vi "optical_1.vi"() -> ()   [LabVIEW 2025]
panel:
  out "Optical saving error":errorcluster
  out "Times between Frames":u32
  in  "STOP ACQUISITION":bool
  out "Optical Frame Out":string
  out "Optical Preview":T1(plugin-control)
  in  "Output Folder":path
  # "Thermal Record"
  # "(Enter \"28\")"
  # "^ append to base data folder \"...\\test_n\\raw\" for nth recording"
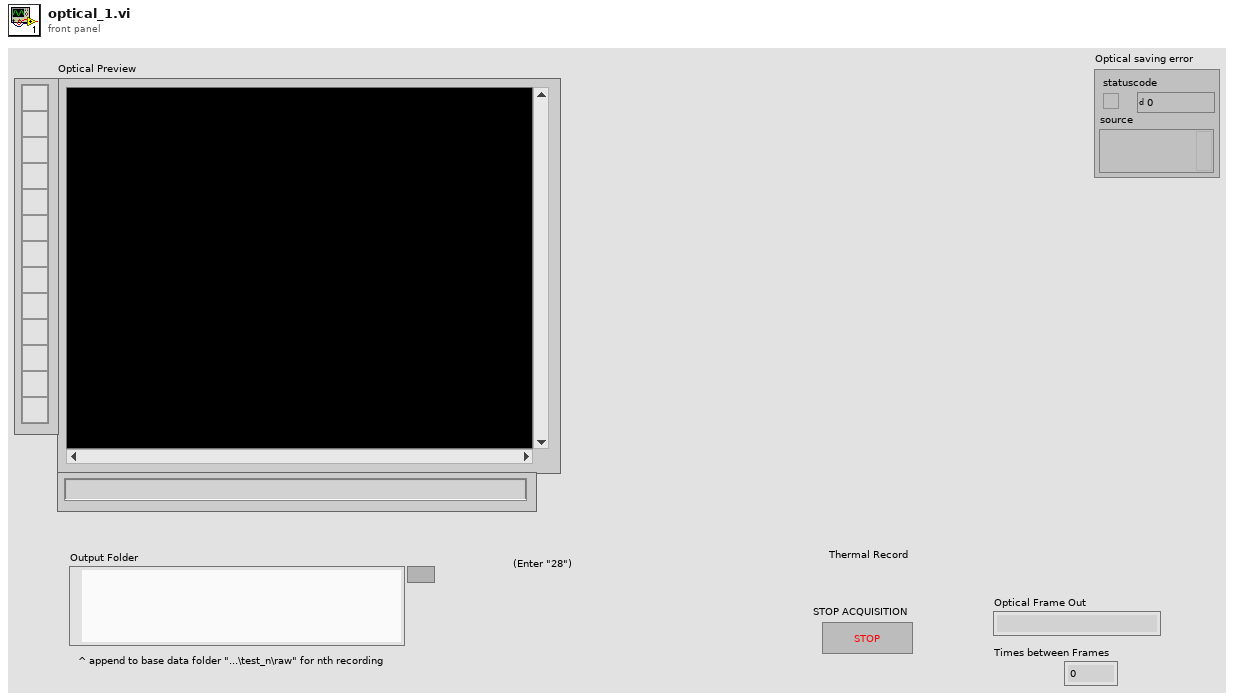
[diagram p1: front panel]
types:
  T1 = typedef "IMAQ Image.ctl" = refnum<image>
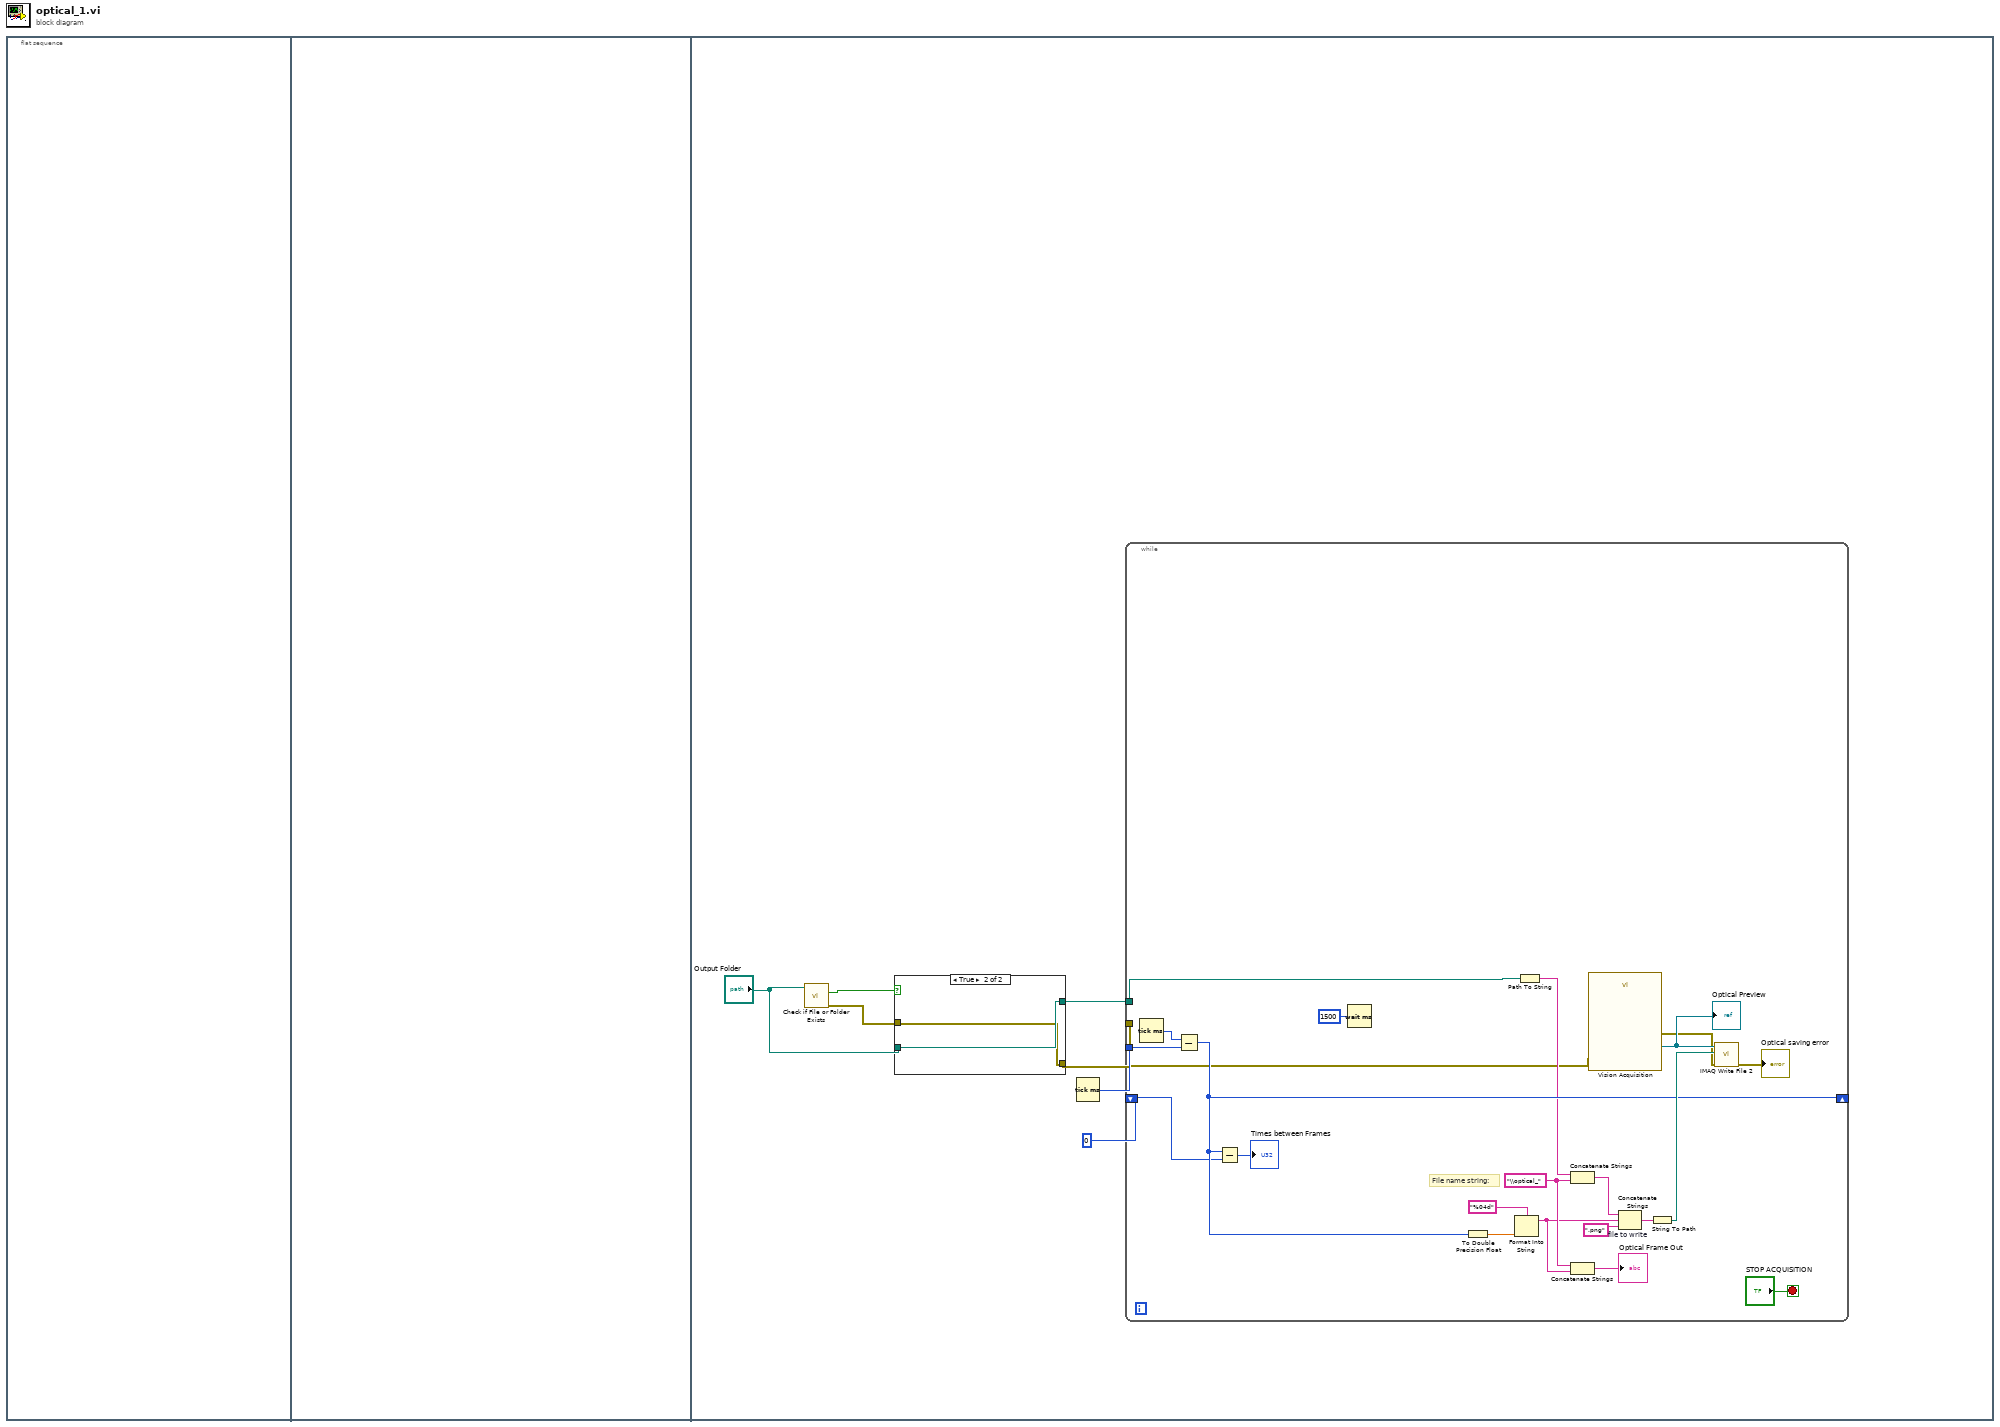
[diagram p0: block diagram]
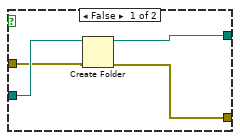
[diagram p2: hidden frame]
diagram:
  n1 = flat-sequence {
    frame #0 {
    }
    frame #1 {
    }
    frame #2 {
      n2 = call <vilib>:"Check if File or Folder Exists.vi"("path"="Output Folder") -> ("error out"=w2:errorcluster, "file or folder exists?"=w5:bool)  [unwired: 8 in, 1 out]
      n3 = case shown="True" w5 {
        tunnel: "Output Folder" -> [w11 w13]
        tunnel: [w10 w13] -> w3
        tunnel: w2 -> [w9 w12]
        tunnel: [w8 w12] -> w1
        frame False {
          n4 = Create Folder(path (use dialog)=w11, error in=w9) -> (created path=w10:path, error out=w8:errorcluster)  [unwired: 1 in, 1 out]
        }
        frame True {
        }
      }
      n5 = Tick Count (ms)() -> (millisecond timer value=w7:u32)
      n6 = while {
        tunnel: w7 -> [w22]
        shift-right: [w21] -> _
        shift-left: u32 0 -> [w20]
        tunnel: w3 -> [w16]
        tunnel: w1 -> [w17]
        stop <- "STOP ACQUISITION" stop-if-true
        w31 = "\\optical_" ("string")
        # "File name string:"
        n7 = Tick Count (ms)() -> (millisecond timer value=w23:u32)
        n8 = Subtract(x=w23, y=w22) -> (x-y=w21:u32)
        n9 = Subtract(x=w21, y=w20) -> (x-y=→"Times between Frames":u32)
        n10 = Wait (ms)(milliseconds to wait=u32 1500) -> ()  [unwired: 1 out]
        n11 = To Double Precision Float(number=w21) -> (double precision float=w29:dbl)
        n12 = Format Into String(format string="%04d" ("time format string (%c)"), w29) -> (resulting string=w27:string)  [unwired: 2 in, 1 out]
        n13 = Path To String(path=w16) -> (string=w18:string)
        n14 = Concatenate Strings(w18, w31) -> (w32:string)
        n15 = Concatenate Strings(w31, w27) -> (→"Optical Frame Out":string)
        n16 = call "Vision Acquisition"("error in"=w17) -> ("Image Out"=w35:T1, "error out"=w15:errorcluster)  [unwired: 25 in]
        "Optical Preview" <- w35
        n17 = Concatenate Strings "file to write"(w32, w27, ".png" ("string")) -> (w34:string)
        n18 = String To Path(string=w34) -> (path=w28:path)
        n19 = call-poly "IMAQ Write File 2"("error in (no error)"=w15, "File Path"=w28, "Image"=w35) -> ("error out"=→"Optical saving error":errorcluster)  [unwired: 7 in, 1 out]
      }
    }
  }
